vi "Gen_TrajLib_Doc_Enum.vi"() -> ()   [LabVIEW 2019]
doc: "Generates and HTML file with the Description of every class, library, ctl, and vi in every open project. Creates separate documents for each library and virtual folder , and links to the top level document. In addition, for every VI shows connector pane. Saves the HTML file in folder <project folder>\\<project name> Documentation\\Documentation.html. erases previous content if any. \nDoes not create documentation for Documentation folder in project if exists. Does not create documentation for packed libraries in the project."
uses:
  Doc_Builder_SubVI/FileAndPath.ctl
  <vilib>/Utility/NIReport.llb/NI_report.lvclass
panel:
  out "Finish Processed":bool
  out "ParamFoundBits":u32
  out "application name":string
  out "Cmd Line Read Error":errorcluster
  out "arguments":string[](array[string])
  in  "Finish":bool
  out "Full Library Path":path
  out "Current Section":string
  out "File Index":i32
  out "File Count":i32
  in  "stop":bool
  out "Full Input File Name":path
  in  "GO":bool
  in  "Documentation Path":path=path "../HTML_Build_Work/Temp"
  in  "Library Path":path=path "../../FRC_LV_Trajectory_Library/Enum"
  out "Full Doc Path":path
  # "DOCUMENT ENUM DEFINITIONS"
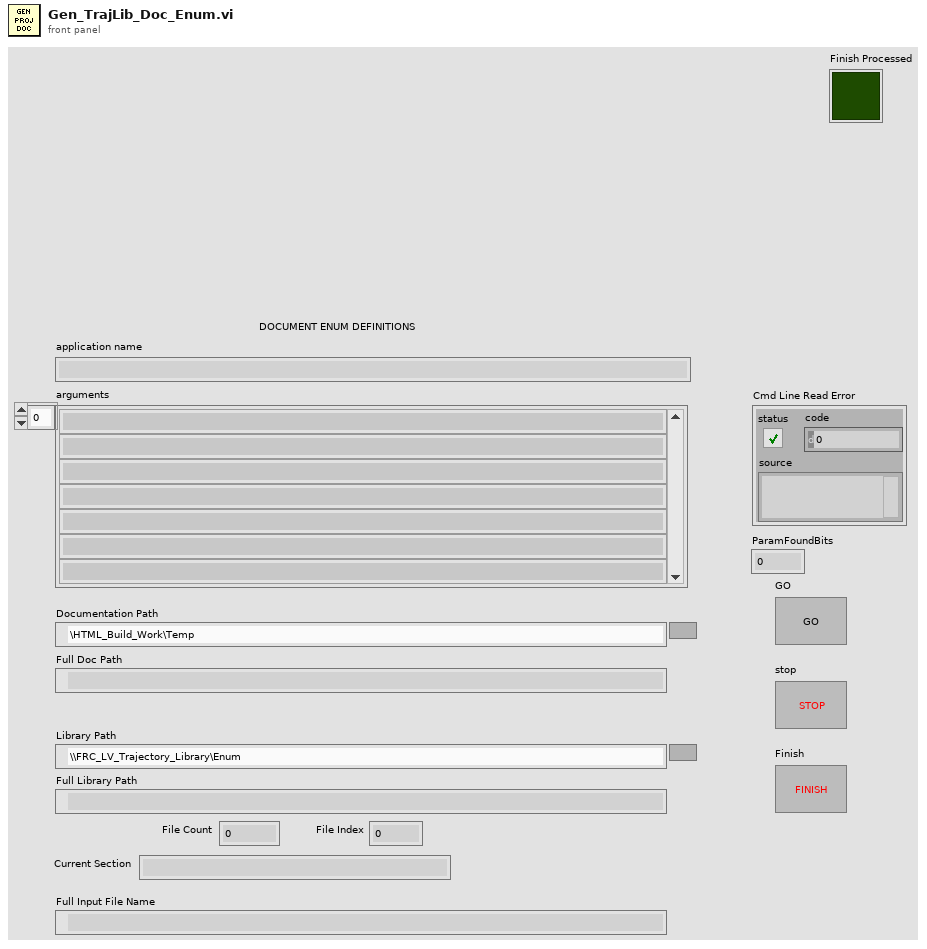
[diagram p1: front panel]
types:
  T1 = typedef "FileAndPath.ctl" = cluster{"FileName":string, "Library Path":path}
  T2 = enum16{"Standard Report", "HTML", "Word", "Excel"}
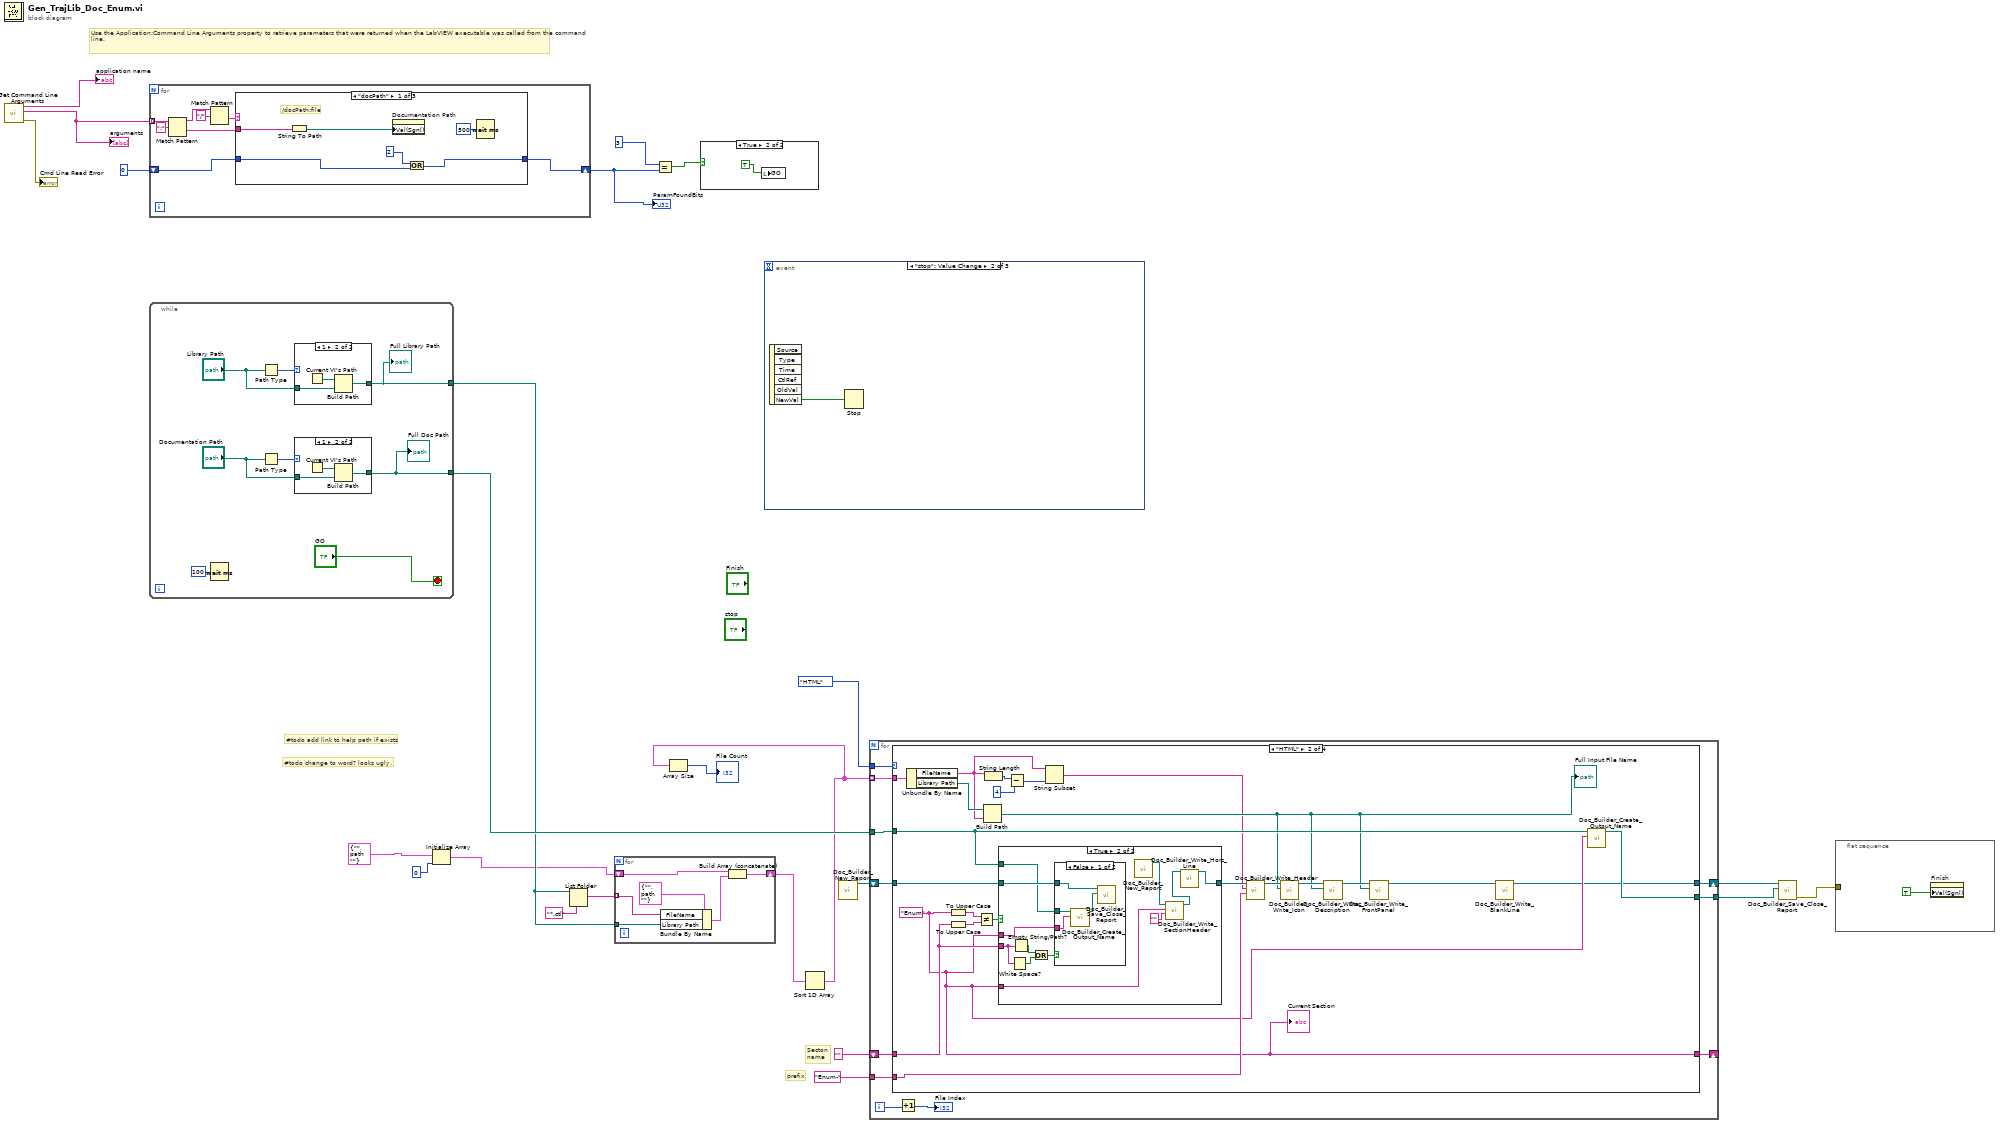
[diagram p0: block diagram]
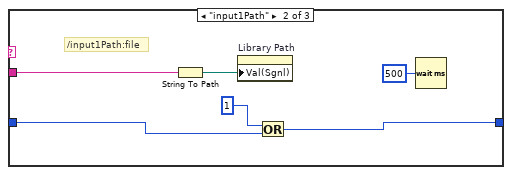
[diagram p3: hidden frame]
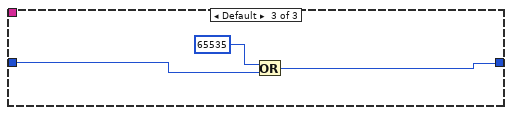
[diagram p4: hidden frame]
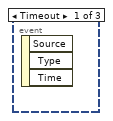
[diagram p5: hidden frame]
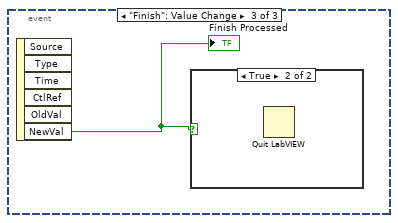
[diagram p6: hidden frame]
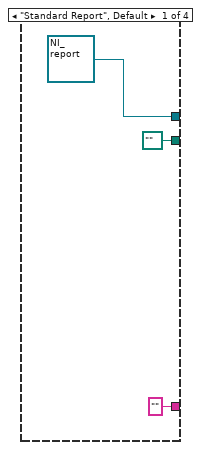
[diagram p10: hidden frame]
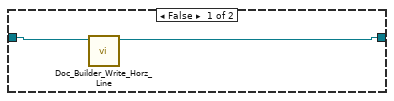
[diagram p11: hidden frame]
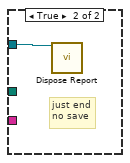
[diagram p12: hidden frame]
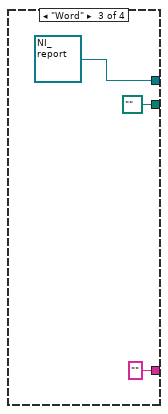
[diagram p13: hidden frame]
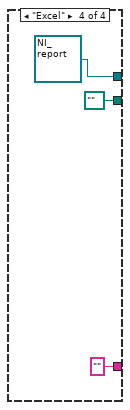
[diagram p14: hidden frame]
diagram:
  # "Use the Application:Command Line Arguments property to retrieve parameters that were returned when the LabVIEW executable was called from the command line."
  # "Secton \nname"
  # "prefix"
  # "#todo change to word? looks ugly."
  # "#todo add link to help path if exists"
  n1 = call <vilib>:"Get Command Line Arguments.vi"() -> ("error out"=→"Cmd Line Read Error":errorcluster, "arguments"=w4:string[], "application name"=→"application name":string)  [unwired: 9 in]
  "arguments" <- w4
  n2 = while {
    tunnel: [w26] -> w22
    tunnel: [w25] -> w18
    stop <- "GO" stop-if-true
    n3 = Wait (ms)(milliseconds to wait=u32 100) -> ()  [unwired: 1 out]
    n4 = Path Type(1:"Library Path") -> (0:w29:i16)
    n5 = Path Type(1:"Documentation Path") -> (0:w30:i16)
    n6 = case shown="1" w29 {
      tunnel: [w33 w35] -> w25
      tunnel: "Library Path" -> [w33 w34]
      frame 0, Default {
      }
      frame 1 {
        n7 = Current VI's Path() -> (path=w36:path)
        n8 = Build Path(base path=w36, name or relative path=w34) -> (appended path=w35:path)
      }
    }
    "Full Library Path" <- w25
    n9 = case shown="1" w30 {
      tunnel: [w37 w39] -> w26
      tunnel: "Documentation Path" -> [w37 w38]
      frame 0, Default {
      }
      frame 1 {
        n10 = Current VI's Path() -> (path=w40:path)
        n11 = Build Path(base path=w40, name or relative path=w38) -> (appended path=w39:path)
      }
    }
    "Full Doc Path" <- w26
  }
  n12 = for {
    tunnel: w4 -> [w47] mode=indexing
    shift-right: [w41] -> w2
    shift-left: u32 0 -> [w42]
    n13 = Match Pattern(string=w47, regular expression=":") -> (before substring=w45:string, after substring=w46:string)  [unwired: 3 out]
    n14 = Match Pattern(string=w45, regular expression="/") -> (after substring=w43:string)  [unwired: 4 out]
    n15 = case shown="\"docPath\"" w43 {
      tunnel: w46 -> [w54 w60 _]
      tunnel: [w51 w58 w61] -> w41
      tunnel: w42 -> [w52 w59 w62]
      frame "docPath" {
        # "/docPath:file"
        n16 = String To Path(string=w54) -> (path=w49:path)
        n17 = property on="Documentation Path" class="Path"("Val(Sgnl)"=w49) -> ()  [unwired: 2 in, 2 out]
        n18 = Or(x=u32 2, y=w52) -> (x .or. y?=w51:u32)
        n19 = Wait (ms)(milliseconds to wait=u32 500) -> ()  [unwired: 1 out]
      }
      frame "input1Path" {
        # "/input1Path:file"
        n20 = String To Path(string=w60) -> (path=w55:path)
        n21 = property on="Library Path" class="Path"("Val(Sgnl)"=w55) -> ()  [unwired: 2 in, 2 out]
        n22 = Or(x=u32 1, y=w59) -> (x .or. y?=w58:u32)
        n23 = Wait (ms)(milliseconds to wait=u32 500) -> ()  [unwired: 1 out]
      }
      frame Default {
        n24 = Or(x=u32 65535, y=w62) -> (x .or. y?=w61:u32)
      }
    }
  }
  "ParamFoundBits" <- w2
  n25 = Initialize Array(T1 {"FileName"="", "Library Path"=path ""} ("FileAndPath"), 0 ("dimension size")) -> (w16:T1[])
  n26 = List Folder(path=w18, pattern="*.ctl") -> (filenames=w19:string[])  [unwired: 2 in, 3 out]
  n27 = for {
    tunnel: w19 -> [w69] mode=indexing
    tunnel: w18 -> [w68]
    shift-right: [w67] -> w9
    shift-left: w16 -> [w66]
    n28 = Bundle By Name(cluster=T1 {"FileName"="", "Library Path"=path ""} ("FileAndPath"), "FileName"=w69, "Library Path"=w68) -> (w64:T1)
    n29 = Build Array (concatenate)(w66, w64) -> (w67:T1[])
  }
  n30 = Equal?(x=u32 3, y=w2) -> (x = y?=w6:bool)
  n31 = case shown="True" w6 {
    frame False {
    }
    frame True {
      n32 = local write "GO"(TRUE ("GO")) -> ()
    }
  }
  n33 = event shown="[1] \"stop\": Value Change" {
    selector: _ -> [_ _ _]
    dyn-events: _ -> [_ _ _]
    timeout: _ -> [_ _ _]
    event Timeout {
      n34 = event-data() -> ()  [unwired: 1 in, 3 out]
    }
    event "stop": Value Change {
      n35 = event-data() -> ("NewVal"=w71:bool)  [unwired: 1 in, 5 out]
      n36 = Stop(stop? (T)=w71) -> ()
    }
    event "Finish": Value Change {
      n37 = event-data() -> ("NewVal"=w72:bool)  [unwired: 1 in, 5 out]
      "Finish Processed" <- w72
      n38 = case shown="True" w72 {
        frame False {
        }
        frame True {
          n39 = Quit LabVIEW() -> ()  [unwired: 1 in]
        }
      }
    }
  }
  n40 = Sort 1D Array(array=w9) -> (sorted array=w14:T1[])
  n41 = Array Size(array=w14) -> (size(s)=→"File Count":i32)
  n42 = call "Doc_Builder_New_Report.vi"() -> ("NI_report out"=w13:refnum<class "NI_report.lvclass">)  [unwired: 11 in]
  n43 = for {
    tunnel: w14 -> [w82] mode=indexing
    tunnel: T2."HTML" ("report type") -> [w83]
    tunnel: w22 -> [w81]
    tunnel: "Enum-" ("string") -> [w78]
    shift-right: [w74] -> w11
    shift-left: w13 -> [w77]
    shift-right: [w73] -> _
    shift-left: "" ("string") -> [w76]
    tunnel: [w75] -> w10
    i -> [w80]
    n44 = case shown="\"HTML\"" w83 {
      tunnel: w82 -> [_ w104 _ _]
      tunnel: w81 -> [_ w95 _ _]
      tunnel: w78 -> [_ w92 _ _]
      tunnel: w77 -> [_ w99 _ _]
      tunnel: w76 -> [_ w96 _ _]
      tunnel: [path "" ("Full Report Name") w97 path "" ("Full Report Name") path "" ("Full Report Name")] -> w75
      tunnel: [refnum<class "NI_report.lvclass"> refnum ("report out") w87 refnum<class "NI_report.lvclass"> refnum ("report out") refnum<class "NI_report.lvclass"> refnum ("report out")] -> w74
      tunnel: ["" ("FileName") w89 "" ("FileName") "" ("FileName")] -> w73
      frame "Standard Report", Default {
      }
      frame "HTML" {
        w89 = "Enum" ("string")
        n45 = Unbundle By Name(w104) -> ("FileName"=w102:string, "Library Path"=w103:path)
        n46 = To Upper Case(1:w89) -> (0:w101:string)
        n47 = To Upper Case(1:w96) -> (0:w100:string)
        n48 = Not Equal?(x=w101, y=w100) -> (x != y?=w90:bool)
        n49 = Build Path(base path=w103, name or relative path=w102) -> (appended path=w93:path)
        "Full Input File Name" <- w93
        n50 = String Length(string=w102) -> (length=w109:i32)
        n51 = case shown="True" w90 {
          tunnel: w99 -> [w111 w120]
          tunnel: [w110 w117] -> w98
          tunnel: w96 -> [_ w118]
          tunnel: w95 -> [_ w119]
          tunnel: w89 -> [_ w114]
          tunnel: w89 -> [_ w113]
          frame False {
            n52 = call "Doc_Builder_Write_Horz_Line.vi"("NI_report in"=w111) -> ("NI_report out"=w110:refnum<class "NI_report.lvclass">)  [unwired: 10 in]
          }
          frame True {
            n53 = White Space?(1:w118) -> (0:w122:bool)
            n54 = Empty String/Path?(string/path=w118) -> (empty?=w121:bool)
            n55 = Or(x=w121, y=w122) -> (x .or. y?=w123:bool)
            n56 = case shown="False" w123 {
              tunnel: w120 -> [w127 w128]
              tunnel: w119 -> [w126 _]
              tunnel: w113 -> [w125 _]
              frame False {
                n57 = call "Doc_Builder_Create_Output_Name.vi"("Section Name"=w125, "Path"=w126) -> ("Full Report Name"=w124:path)  [unwired: 9 in]
                n58 = call "Doc_Builder_Save_Close_Report.vi"("appended path"=w124, "NI_report in"=w127) -> ()  [unwired: 9 in, 1 out]
              }
              frame True {
                # "just end\nno save"
                n59 = call-dynamic "Dispose Report.vi"("report in"=w128) -> ()  [unwired: 14 in, 1 out]
              }
            }
            n60 = call "Doc_Builder_New_Report.vi"() -> ("NI_report out"=w116:refnum<class "NI_report.lvclass">)  [unwired: 11 in]
            n61 = call "Doc_Builder_Write_SectionHeader.vi"("Prefix String"="", "Section Name"=w114, "NI_report in"=w116) -> ("NI_report out"=w115:refnum<class "NI_report.lvclass">)  [unwired: 8 in]
            n62 = call "Doc_Builder_Write_Horz_Line.vi"("NI_report in"=w115) -> ("NI_report out"=w117:refnum<class "NI_report.lvclass">)  [unwired: 10 in]
          }
        }
        n63 = Subtract(x=w109, y=4) -> (x-y=w107:i32)
        n64 = String Subset(string=w102, length (rest)=w107) -> (substring=w91:string)  [unwired: 1 in]
        n65 = call "Doc_Builder_Write_Header.vi"("Prefix String"=w92, "Item Name"=w91, "NI_report in"=w98) -> ("NI_report out"=w106:refnum<class "NI_report.lvclass">)  [unwired: 8 in]
        n66 = call "Doc_Builder_Write_Icon.vi"("Input Item file path"=w93, "NI_report in"=w106) -> ("NI_report out"=w105:refnum<class "NI_report.lvclass">)  [unwired: 9 in]
        n67 = call "Doc_Builder_Write_Description.vi"("input item file path"=w93, "NI_report in"=w105) -> ("NI_report out"=w94:refnum<class "NI_report.lvclass">)  [unwired: 9 in]
        n68 = call "Doc_Builder_Write_FrontPanel.vi"("input item file path"=w93, "NI_report in"=w94) -> ("NI_report out"=w88:refnum<class "NI_report.lvclass">)  [unwired: 9 in]
        n69 = call "Doc_Builder_Write_BlankLine.vi"("NI_report in"=w88) -> ("NI_report out"=w87:refnum<class "NI_report.lvclass">)  [unwired: 10 in]
        n70 = call "Doc_Builder_Create_Output_Name.vi"("Section Name"=w89, "Path"=w95) -> ("Full Report Name"=w97:path)  [unwired: 9 in]
        "Current Section" <- w89
      }
      frame "Word" {
      }
      frame "Excel" {
      }
    }
    n71 = Increment(x=w80) -> (x+1=→"File Index":i32)
  }
  n72 = call "Doc_Builder_Save_Close_Report.vi"("appended path"=w10, "NI_report in"=w11) -> ("error out"=w1:errorcluster)  [unwired: 9 in]
  n73 = flat-sequence {
    tunnel: w1 -> [_]
    frame #0 {
      n74 = property on="Finish" class="Bool (strict)"("Val(Sgnl)"=TRUE) -> ()  [unwired: 2 in, 2 out]
    }
  }
